vi "Unregister.vi"(0 "BroadcastRegistry In":T1, 5 "Broadcast":string, 7 "SourceCSM":string, 9 "API":string="api", 11 "TargetCSM":string) -> (4 "BroadcastRegistry Out":T1)   [LabVIEW 2017, in "Communicable State Machine.lvlib"]
doc: "### Unregister.vi\n\n-- <b>Controls</b> --\n- <b>BroadcastRegistry in</b>:\n- <b>Status</b>:\n- <b>Source</b>:\n- <b>api</b>:\n- <b>Target</b>:\n\n-- <b>Indicators</b> --\n- <b>BroadcastRegistry out</b>:"
uses:
  Communicable State Machine.lvlib
  BroadcastRegistry.ctl
  BroadcastRegistry-Value.ctl
  AdvanceAPI/CSM - Broadcast Message Type.ctl
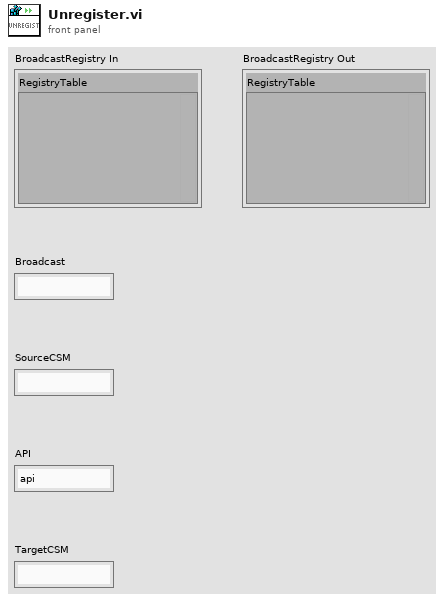
[diagram p1: front panel]
types:
  T1 = typedef "Communicable State Machine.lvlib/BroadcastRegistry.ctl" = cluster{"RegistryTable":variant}
  T2 = typedef "Communicable State Machine.lvlib/BroadcastRegistry-Value.ctl" = cluster{"Name":string, "Register Type":T3}
  T3 = typedef "Communicable State Machine.lvlib/CSM - Broadcast Message Type.ctl" = enum16{"<Null>", "Status", "Interrupt"}
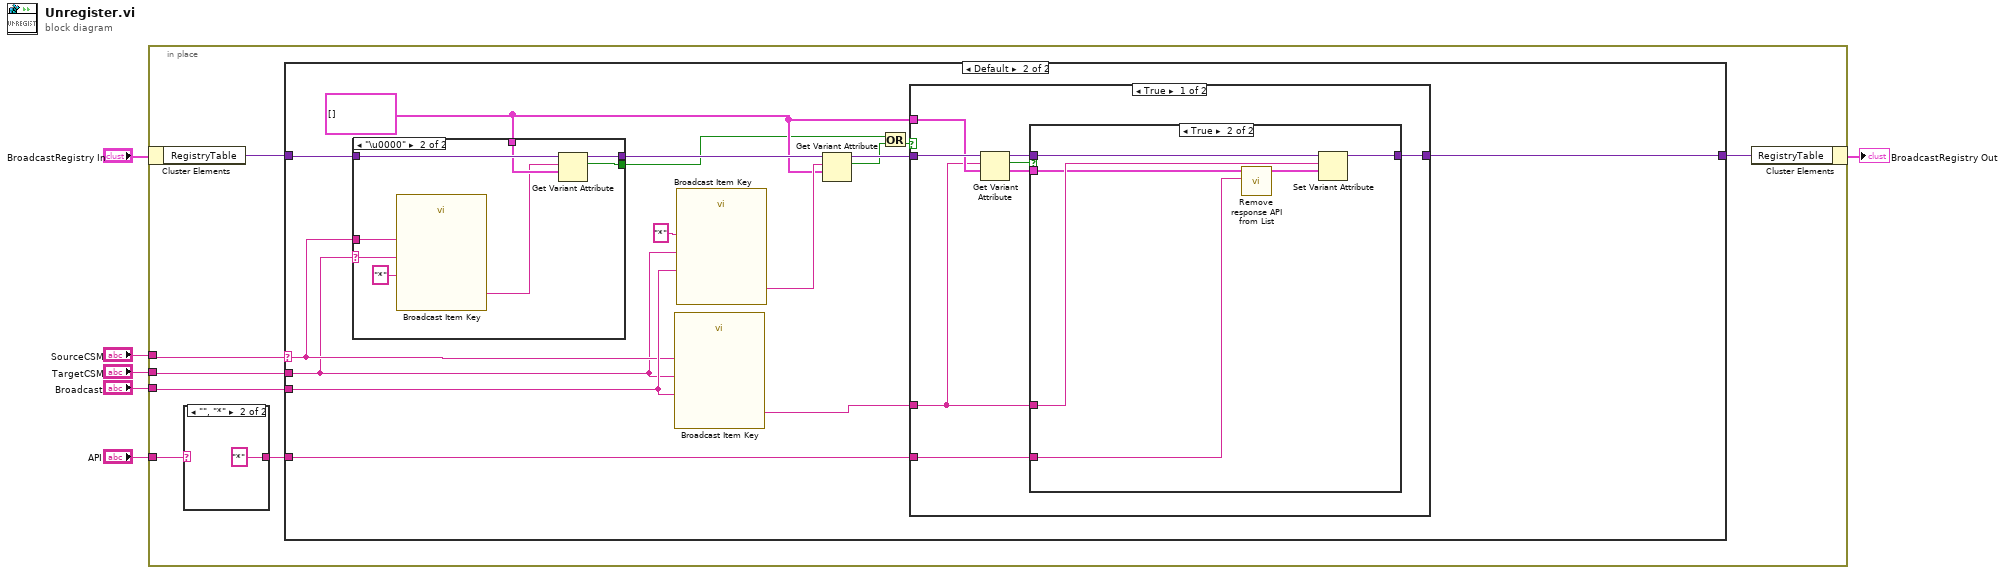
[diagram p0: block diagram]
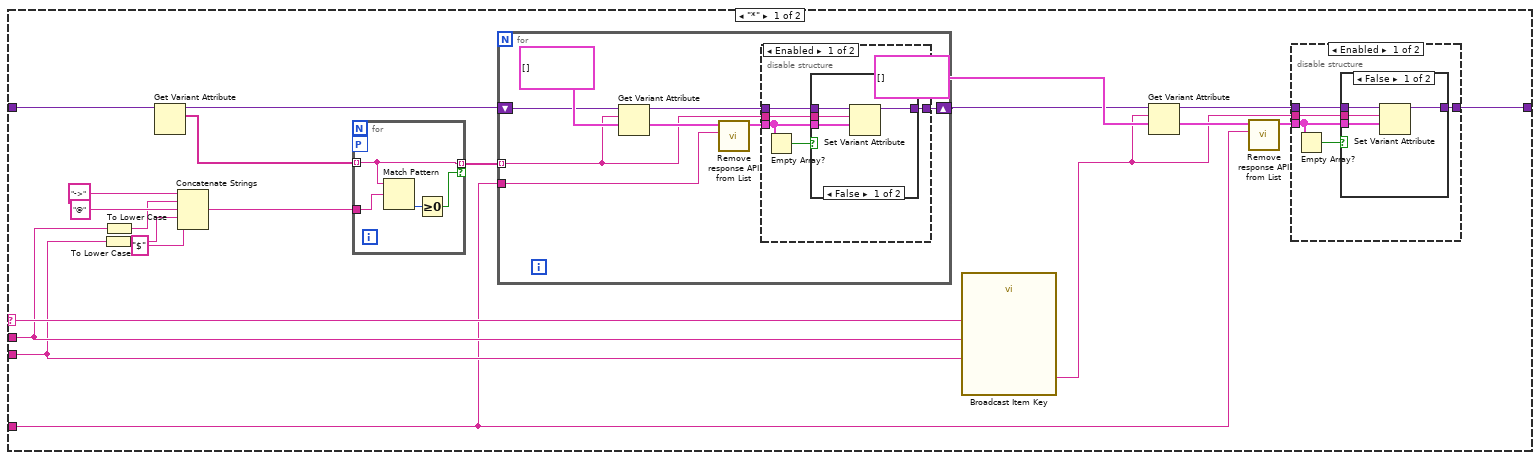
[diagram p2: hidden frame]
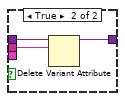
[diagram p3: hidden frame]
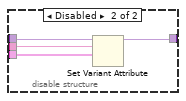
[diagram p4: hidden frame]
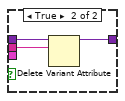
[diagram p5: hidden frame]
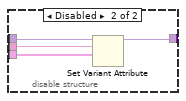
[diagram p6: hidden frame]
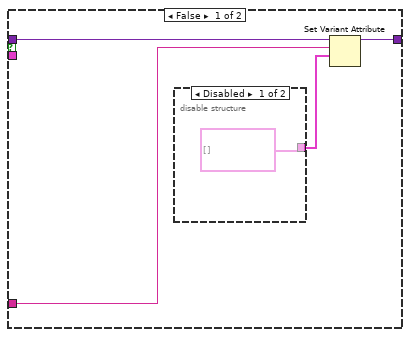
[diagram p8: hidden frame]
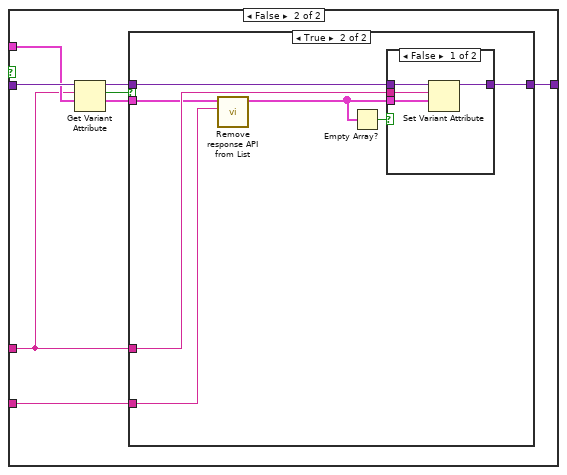
[diagram p10: hidden frame]
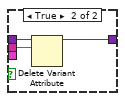
[diagram p12: hidden frame]
diagram:
  n1 = in-place {
    in-place-border: "Broadcast" -> [w9]
    in-place-border: "TargetCSM" -> [w10]
    in-place-border: "SourceCSM" -> [w11]
    in-place-border: "API" -> [w8]
    n2 = in-place-cluster #1("BroadcastRegistry In") -> ("RegistryTable"=w13:variant)
    n3 = case shown="\"\", \"*\"" w8 {
      selector: w8 -> [w145 _]
      tunnel: [w145 "*"] -> w7
      frame Default {
      }
      frame "", "*" {
      }
    }
    n4 = case shown="Default" w11 {
      selector: w11 -> [w34 w85]
      tunnel: w13 -> [w26 w83]
      tunnel: [w17 w93] -> w12
      tunnel: w10 -> [w25 w84]
      tunnel: w9 -> [w24 w88]
      tunnel: w7 -> [w14 w86]
      frame "*" {
        n5 = To Lower Case(string=w24) -> (all lower case string=w27:string)
        n6 = To Lower Case(string=w25) -> (all lower case string=w29:string)
        n7 = Get Variant Attribute(Variant=w26) -> (duplicate Variant=w33:variant, names=w32:string[])  [unwired: 3 in, 2 out]
        n8 = Concatenate Strings("->" ("string"), w29, "@" ("string"), w27, "$" ("string")) -> (w22:string)
        n9 = for {
          tunnel: w32 -> [w78] mode=indexing
          tunnel: [w78] -> w28 mode=indexing if=w75
          tunnel: w22 -> [w77]
          workers-P: _ -> [_]
          n10 = Match Pattern(string=w78, regular expression=w77) -> (offset past match=w76:i32)  [unwired: 1 in, 3 out]
          n11 = Greater Or Equal To 0?(x=w76) -> (x >= 0?=w75:bool)
        }
        n12 = for {
          shift-right: [w54] -> w16
          shift-left: w33 -> [w51]
          tunnel: w28 -> [w52] mode=indexing
          tunnel: w14 -> [w57]
          n13 = Get Variant Attribute(Variant=w51, name=w52, default value (empty Variant)=T2[] [] ("string")) -> (duplicate Variant=w55:variant, value=w56:T2[])  [unwired: 1 in, 2 out]
          n14 = call "Remove response API from List.vi"("API"=w57, "Output Cluster In"=w56) -> ("Output Cluster Out"=w53:T2[])  [unwired: 9 in]
          n15 = disable-structure shown="Enabled" {
            disable-tunnel: w55 -> [w62 w73]
            disable-tunnel: [w61 w71] -> w54
            disable-tunnel: w53 -> [w60 w72]
            disable-tunnel: w52 -> [w59 w74]
            frame Enabled {
              n16 = Empty Array?(array=w60) -> (empty?=w63:bool)
              n17 = case shown="False" w63 {
                tunnel: [w67 w70] -> w61
                tunnel: w62 -> [w66 w69]
                tunnel: w60 -> [w65 _]
                tunnel: w59 -> [w64 w68]
                frame False {
                  n18 = Set Variant Attribute(Variant=w66, name=w64, value=w65) -> (Variant out=w67:variant)  [unwired: 1 in, 2 out]
                }
                frame True {
                  n19 = Delete Variant Attribute(6:w68, 7:w69) -> (3:w70:variant)  [unwired: 1 in, 2 out]
                }
              }
            }
            frame Disabled {
              n20 = Set Variant Attribute(Variant=w73, name=w74, value=w72) -> (Variant out=w71:variant)  [unwired: 1 in, 2 out]
            }
          }
        }
        n21 = call "Broadcast Item Key.vi"("Status"=w24, "Target"=w25, "Source"=w34) -> ("Key"=w15:string)  [unwired: 2 in]
        n22 = Get Variant Attribute(Variant=w16, name=w15, default value (empty Variant)=T2[] [] ("string")) -> (duplicate Variant=w19:variant, value=w20:T2[])  [unwired: 1 in, 2 out]
        n23 = call "Remove response API from List.vi"("API"=w14, "Output Cluster In"=w20) -> ("Output Cluster Out"=w18:T2[])  [unwired: 9 in]
        n24 = disable-structure shown="Enabled" {
          disable-tunnel: w19 -> [w38 w49]
          disable-tunnel: [w37 w47] -> w17
          disable-tunnel: w18 -> [w36 w48]
          disable-tunnel: w15 -> [w35 w50]
          frame Enabled {
            n25 = Empty Array?(array=w36) -> (empty?=w39:bool)
            n26 = case shown="False" w39 {
              tunnel: [w43 w46] -> w37
              tunnel: w38 -> [w42 w45]
              tunnel: w36 -> [w41 _]
              tunnel: w35 -> [w40 w44]
              frame False {
                n27 = Set Variant Attribute(Variant=w42, name=w40, value=w41) -> (Variant out=w43:variant)  [unwired: 1 in, 2 out]
              }
              frame True {
                n28 = Delete Variant Attribute(6:w44, 7:w45) -> (3:w46:variant)  [unwired: 1 in, 2 out]
              }
            }
          }
          frame Disabled {
            n29 = Set Variant Attribute(Variant=w49, name=w50, value=w48) -> (Variant out=w47:variant)  [unwired: 1 in, 2 out]
          }
        }
      }
      frame Default {
        w81 = T2[] [] ("output cluster")
        n30 = case shown="\"\"" w84 {
          selector: w84 -> [_ w100]
          tunnel: w85 -> [_ w101]
          tunnel: w83 -> [w94 w99]
          tunnel: [w94 w98] -> w82
          tunnel: w81 -> [_ w97]
          tunnel: [_ w95] -> w79
          frame Default {
          }
          frame "\u0000" {
            n31 = call "Broadcast Item Key.vi"("Status"="*", "Target"=w100, "Source"=w101) -> ("Key"=w96:string)  [unwired: 2 in]
            n32 = Get Variant Attribute(Variant=w99, name=w96, default value (empty Variant)=w97) -> (duplicate Variant=w98:variant, found=w95:bool)  [unwired: 1 in, 2 out]
          }
        }
        n33 = call "Broadcast Item Key.vi"("Status"=w88, "Target"=w84, "Source"=w85) -> ("Key"=w87:string)  [unwired: 2 in]
        n34 = call "Broadcast Item Key.vi"("Status"=w88, "Target"=w84, "Source"="*") -> ("Key"=w90:string)  [unwired: 2 in]
        n35 = Get Variant Attribute(Variant=w82, name=w90, default value (empty Variant)=w81) -> (duplicate Variant=w91:variant, found=w89:bool)  [unwired: 1 in, 2 out]
        n36 = Or(x=w79, y=w89) -> (x .or. y?=w80:bool)
        n37 = case shown="True" w80 {
          tunnel: [w110 w129] -> w93
          tunnel: w91 -> [w109 w128]
          tunnel: w87 -> [w106 w125]
          tunnel: w81 -> [w107 w126]
          tunnel: w86 -> [w103 w123]
          frame True {
            n38 = Get Variant Attribute(Variant=w109, name=w106, default value (empty Variant)=w107) -> (duplicate Variant=w108:variant, found=w105:bool, value=w104:T2[])  [unwired: 1 in, 1 out]
            n39 = case shown="True" w105 {
              tunnel: [w114 w121] -> w110
              tunnel: w108 -> [w112 w120]
              tunnel: w106 -> [w111 w119]
              tunnel: w104 -> [_ w117]
              tunnel: w103 -> [_ w118]
              frame False {
                n40 = disable-structure shown="Disabled" {
                  disable-tunnel: [T2[] [] ("output cluster") _] -> w113
                  frame Disabled {
                  }
                  frame Enabled {
                  }
                }
                n41 = Set Variant Attribute(Variant=w112, name=w111, value=w113) -> (Variant out=w114:variant)  [unwired: 1 in, 2 out]
              }
              frame True {
                n42 = call "Remove response API from List.vi"("API"=w118, "Output Cluster In"=w117) -> ("Output Cluster Out"=w116:T2[])  [unwired: 9 in]
                n43 = Set Variant Attribute(Variant=w120, name=w119, value=w116) -> (Variant out=w121:variant)  [unwired: 1 in, 2 out]
              }
            }
          }
          frame False {
            n44 = Get Variant Attribute(Variant=w128, name=w125, default value (empty Variant)=w126) -> (duplicate Variant=w127:variant, found=w122:bool, value=w124:T2[])  [unwired: 1 in, 1 out]
            n45 = case shown="True" w122 {
              tunnel: [w130 w137] -> w129
              tunnel: w127 -> [w130 w136]
              tunnel: w125 -> [_ w135]
              tunnel: w124 -> [_ w132]
              tunnel: w123 -> [_ w131]
              frame False {
              }
              frame True {
                n46 = call "Remove response API from List.vi"("API"=w131, "Output Cluster In"=w132) -> ("Output Cluster Out"=w134:T2[])  [unwired: 9 in]
                n47 = Empty Array?(array=w134) -> (empty?=w133:bool)
                n48 = case shown="False" w133 {
                  tunnel: [w141 w143] -> w137
                  tunnel: w136 -> [w140 w144]
                  tunnel: w135 -> [w139 w142]
                  tunnel: w134 -> [w138 _]
                  frame False {
                    n49 = Set Variant Attribute(Variant=w140, name=w139, value=w138) -> (Variant out=w141:variant)  [unwired: 1 in, 2 out]
                  }
                  frame True {
                    n50 = Delete Variant Attribute(6:w142, 7:w144) -> (3:w143:variant)  [unwired: 1 in, 2 out]
                  }
                }
              }
            }
          }
        }
      }
    }
    n51 = in-place-cluster #1("RegistryTable"=w12) -> (→"BroadcastRegistry Out":T1)
  }
